vi "VIH Constant - Main INI File.vi"() -> (2 "Main INI File":path, 3 "Section":string)   [LabVIEW 2014]
doc: "::: VI Helpeks :::\nCopyright (c) 2000-2026 Konstantin Shifershteyn. All rights reserved."
panel:
  # "VI Helpeks\nCopyright (c) 2012-2026 Konstantin Shifershteyn"
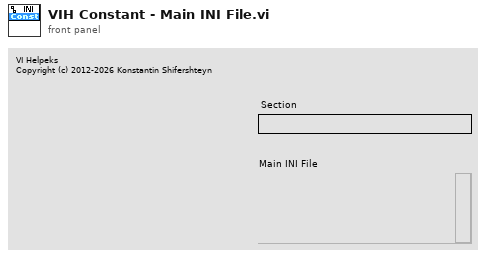
[diagram p1: front panel]
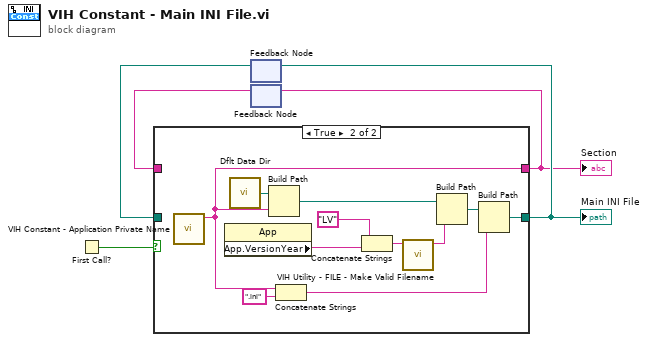
[diagram p0: block diagram]
diagram:
  n1 = First Call?() -> (First Call?: T/F=w5:bool)
  n2 = feedback #1() -> (w4:path)  [unwired: 1 in]
  n3 = feedback #2() -> (w2:string)  [unwired: 1 in]
  n4 = case shown="True" w5 {
    tunnel: [w7 w15] -> w3
    tunnel: w4 -> [w7 _]
    tunnel: [w6 w14] -> w1
    tunnel: w2 -> [w6 _]
    frame False {
    }
    frame True {
      n5 = call "VIH Constant - Application Private Name.vi"() -> ("Name out"=w14:string)  [unwired: 11 in]
      n6 = property class="App"() -> ("App.VersionYear"=w11:string)  [unwired: 2 in, 2 out]
      n7 = call <vilib>:"Dflt Data Dir.vi"() -> ("App:Default Data Directory"=w18:path)
      n8 = Build Path(base path=w18, name or relative path=w14) -> (appended path=w13:path)
      n9 = Concatenate Strings(w14, ".ini" ("string")) -> (w16:string)
      n10 = Concatenate Strings("LV", w11) -> (w9:string)
      n11 = call "VIH Utility - FILE - Make Valid Filename.vi"("File Name in"=w9) -> ("File Name out"=w10:string)  [unwired: 10 in]
      n12 = Build Path(base path=w13, name or relative path=w10) -> (appended path=w12:path)
      n13 = Build Path(base path=w12, name or relative path=w16) -> (appended path=w15:path)
    }
  }
  "Main INI File" <- w3
  "Section" <- w1
  n14 = feedback-in #1(w3) -> ()
  n15 = feedback-in #2(w1) -> ()
